vi "subSetStage.vi"(1 "AxisId":i32=1, 2 "Index":i32=1) -> ()   [LabVIEW 2020]
panel:
  in  "Drive type":u16(ring)=2 items=["DC-Brush"=0, "Stepper Open Loop PMD"=2, "Stepper Closed Loop"=3]
  in  "Resolution":dbl min=0.0 step=0.0001 format="%.6f"
  in  "Resol":bool caption="Full resolution per step/pulse"
  in  "Close":bool caption="Cancel"
  in  "OK":bool
  in  "IncRev":i32=200 caption="Steps/pulses per\nrevolution" min=0
  in  "ratio":dbl=1.0 caption="Gear reduction ratio" min=0.0 step=0.01 format="%.4f"
  in  "pitch":dbl=1.0 caption="Pitch" min=0.0 step=0.1 format="%.4f"
  # "Axis"
  # ": 1"
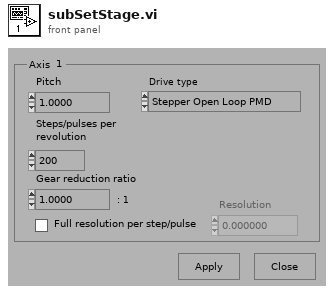
[diagram p1: front panel]
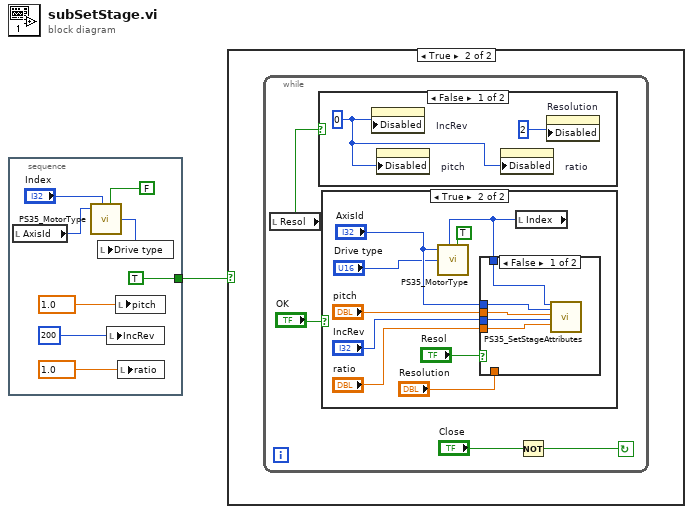
[diagram p0: block diagram]
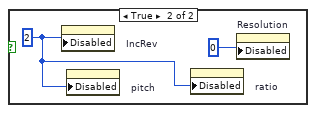
[diagram p3: hidden frame]
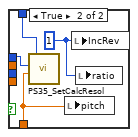
[diagram p5: hidden frame]
diagram:
  n1 = stacked-sequence {
    tunnel: [TRUE ("function")] -> w1
    frame #0 {
      n2 = local read "AxisId"() -> (w7:i32)
      n3 = call "PS35_MotorType.vi"("Axis number"=w7, "Control unit ID"="Index", "function"=FALSE) -> ("Value-Out"=w6:i32)  [unwired: 5 in, 1 out]
      n4 = local write "Drive type"(w6) -> ()
      n5 = local write "IncRev"(200 ("IncRev")) -> ()
      n6 = local write "pitch"(1.0 ("pitch")) -> ()
      n7 = local write "ratio"(1.0 ("ratio")) -> ()
    }
  }
  n8 = case shown="True" w1 {
    frame False {
    }
    frame True {
      n9 = while {
        stop <- w10 continue-if-true
        n10 = local read "Resol"() -> (w12:bool)
        n11 = case shown="False" w12 {
          frame False {
            w14 = u8 0 ("Disabled")
            n12 = property on="IncRev" class="DigNum (strict)"("Disabled"=w14) -> ()  [unwired: 2 in, 2 out]
            n13 = property on="pitch" class="DigNum (strict)"("Disabled"=w14) -> ()  [unwired: 2 in, 2 out]
            n14 = property on="ratio" class="DigNum (strict)"("Disabled"=w14) -> ()  [unwired: 2 in, 2 out]
            n15 = property on="Resolution" class="DigNum (strict)"("Disabled"=u8 2) -> ()  [unwired: 2 in, 2 out]
          }
          frame True {
            w16 = u8 2 ("Disabled")
            n16 = property on="IncRev" class="DigNum (strict)"("Disabled"=w16) -> ()  [unwired: 2 in, 2 out]
            n17 = property on="pitch" class="DigNum (strict)"("Disabled"=w16) -> ()  [unwired: 2 in, 2 out]
            n18 = property on="ratio" class="DigNum (strict)"("Disabled"=w16) -> ()  [unwired: 2 in, 2 out]
            n19 = property on="Resolution" class="DigNum (strict)"("Disabled"=u8 0) -> ()  [unwired: 2 in, 2 out]
          }
        }
        n20 = case shown="True" "OK" {
          frame False {
          }
          frame True {
            n21 = local read "Index"() -> (w18:i32)
            n22 = call "PS35_MotorType.vi"("Axis number"="AxisId", "Control unit ID"=w18, "Value-In"="Drive type", "function"=TRUE) -> ()  [unwired: 4 in, 2 out]
            n23 = case shown="False" "Resol" {
              tunnel: "AxisId" -> [w28 w35]
              tunnel: "pitch" -> [w31 _]
              tunnel: "IncRev" -> [w30 _]
              tunnel: "ratio" -> [w29 _]
              tunnel: "Resolution" -> [_ w34]
              tunnel: w18 -> [w27 w32]
              frame False {
                n24 = call "PS35_SetStageAttributes.vi"("Control unit ID"=w27, "Axis number"=w28, "Pitch"=w31, "IncRev"=w30, "Ratio"=w29) -> ()  [unwired: 14 in, 1 out]
              }
              frame True {
                w33 = u8 1 ("Disabled")
                n25 = call "PS35_SetCalcResol.vi"("dValue"=w34, "Axis number"=w35, "Control unit ID"=w32) -> ()  [unwired: 4 in, 1 out]
                n26 = local write "pitch"(w34) -> ()
                n27 = local write "IncRev"(w33) -> ()
                n28 = local write "ratio"(w33) -> ()
              }
            }
          }
        }
        n29 = Not(x="Close") -> (.not. x?=w10:bool)
      }
    }
  }
